vi "Build Discover Response.vi"(8 "error in":errorcluster, 9 "_meta":string, 10 "capabilities":string, 11 "id":string) -> (0 "error out":errorcluster, 3 "response":string)   [LabVIEW 2020, in "MCP Server.lvlib"]
doc: "Builds the JSON-RPC response to server/discover (MCP 2026-07-28): resultType complete, supportedVersions = all versions of Supported Protocol Versions.vi, the capabilities and _meta from Read Server Info.vi, and the cache hints of Cache Hints.vi for server/discover. id is the JSON text of the request id.\n\nRuns regardless of error in, which is passed through unchanged; the JSONtext errors are not passed on."
uses:
  MCP Server.lvlib
  112a22f7-8e15-46fb-a081-00a3341212e2.vi
  16cc8ae5-8008-4f76-a0d2-c35c9ebad310.vi
  <vilib>/JDP Science/JSONtext/Variant to JSON Text.vi
  <vilib>/JDP Science/JSONtext/LVClass Serializer/JSONtext LVClass Serializer.lvclass
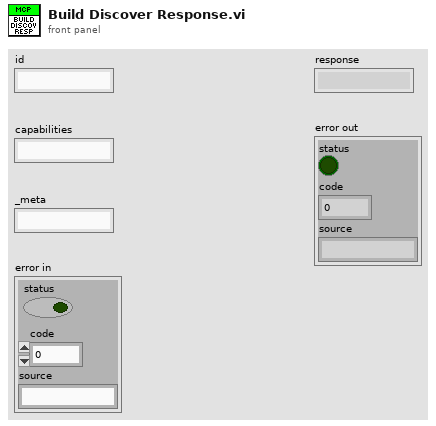
[diagram p1: front panel]
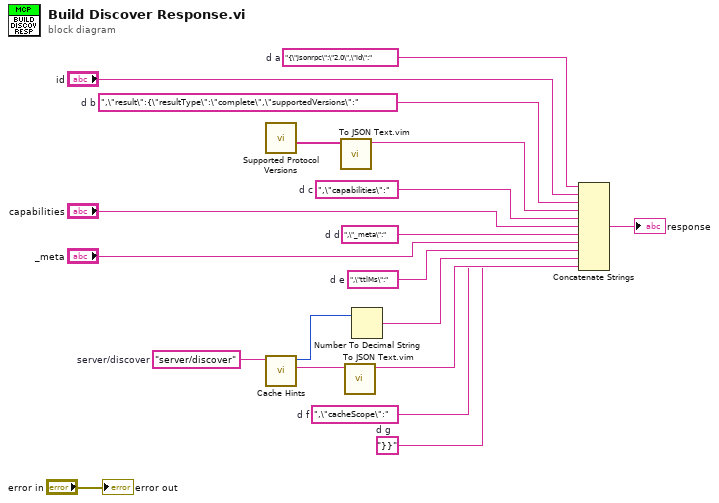
[diagram p0: block diagram]
diagram:
  w12 = "}}"  # d g
  w11 = ",\"cacheScope\":"  # d f
  w10 = ",\"ttlMs\":"  # d e
  w9 = ",\"_meta\":"  # d d
  w8 = ",\"capabilities\":"  # d c
  w7 = ",\"result\":{\"resultType\":\"complete\",\"supportedVersions\":"  # d b
  w6 = "{\"jsonrpc\":\"2.0\",\"id\":"  # d a
  w5 = "server/discover"  # server/discover
  n1 = call "Supported Protocol Versions.vi"() -> ("all versions"=w13:string[])  [unwired: 9 in, 2 out]
  n2 = call "Cache Hints.vi"("method"=w5) -> ("cacheScope"=w14:string, "ttlMs"=w15:i32)  [unwired: 8 in, 1 out]
  n3 = call "To JSON Text.vim"("Anything"=w13) -> ("<JSON>"=w16:string)  [unwired: 9 in, 1 out]
  n4 = call "To JSON Text.vim"("Anything"=w14) -> ("<JSON>"=w17:string)  [unwired: 9 in, 1 out]
  n5 = Number To Decimal String(number=w15) -> (decimal integer string=w18:string)  [unwired: 1 in]
  n6 = Concatenate Strings(w6, "id", w7, w16, w8, "capabilities", w9, "_meta", w10, w18, w11, w17, w12) -> (→"response":string)
  "error out" <- "error in"
